vi "LabVIEW.Service.File_path.vi"(8 "Fehler (Eingang, kein Fehler)":errorcluster, 10 "File name":string, 11 "VI Reference":refnum<vi>) -> (0 "Fehler (Ausgang)":errorcluster, 3 "Dateipfad-Bedienelement":path)   [LabVIEW 2026]
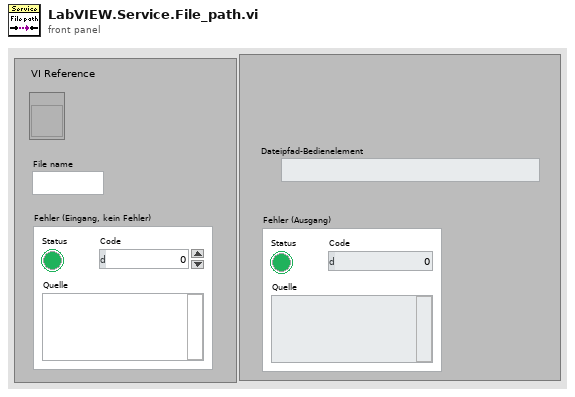
[diagram p1: front panel]
types:
  T1 = enum32{"invalid app kind", "Development System", "Run Time System", "Student Edition", "Embedded LabVIEW", "Evaluation", "Custom"}
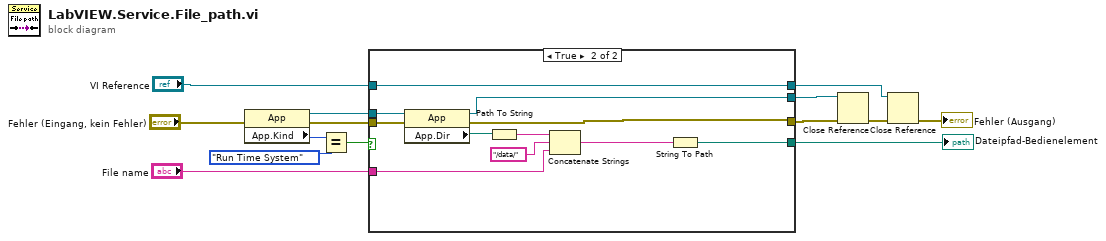
[diagram p0: block diagram]
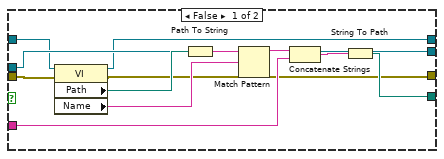
[diagram p2: hidden frame]
diagram:
  n1 = property class="App"(error in="Fehler (Eingang, kein Fehler)") -> (reference out=w9:refnum<vi>, error out=w11:errorcluster, "App.Kind"=w14:T1)  [unwired: 1 in]
  n2 = Equal?(x=w14, y=T1."Run Time System") -> (x = y?=w12:bool)
  n3 = case shown="True" w12 {
    tunnel: w11 -> [w21 w37]
    tunnel: "File name" -> [w20 w33]
    tunnel: [w16 w29] -> w7
    tunnel: [w19 w31] -> w5
    tunnel: w9 -> [w18 w30]
    tunnel: [w18 w28] -> w8
    tunnel: "VI Reference" -> [w17 w27]
    tunnel: [w15 w27] -> w1
    frame False {
      n4 = property class="VI"(reference=w17, error in=w21) -> (reference out=w15:refnum<vi>, error out=w16:errorcluster, "Path"=w26:path, "Name"=w24:string)
      n5 = Path To String(path=w26) -> (string=w25:string)
      n6 = Match Pattern(string=w25, regular expression=w24) -> (before substring=w23:string)  [unwired: 1 in, 3 out]
      n7 = Concatenate Strings(w23, w20) -> (w22:string)
      n8 = String To Path(string=w22) -> (path=w19:path)
    }
    frame True {
      n9 = property class="App"(reference=w30, error in=w37) -> (reference out=w28:refnum<vi>, error out=w29:errorcluster, "App.Dir"=w36:path)
      n10 = Path To String(path=w36) -> (string=w35:string)
      n11 = Concatenate Strings(w35, "/data/" ("Element"), w33) -> (w32:string)
      n12 = String To Path(string=w32) -> (path=w31:path)
    }
  }
  "Dateipfad-Bedienelement" <- w5
  n13 = Close Reference(reference=w8, error in (no error)=w7) -> (error out=w3:errorcluster)
  n14 = Close Reference(reference=w1, error in (no error)=w3) -> (error out=→"Fehler (Ausgang)":errorcluster)
